vi "Alignment Value Change.vi"(8 "error in":errorcluster, 9 "NewVal":T1 items=["left", "center", "right"], 11 "Line Text":refnum<vi>[](array[refnum])) -> (0 "error out":errorcluster)   [LabVIEW 2020]
uses:
  vi.lib/LabVIEW Icon API/lv_icon/Controls/Alignment.ctl
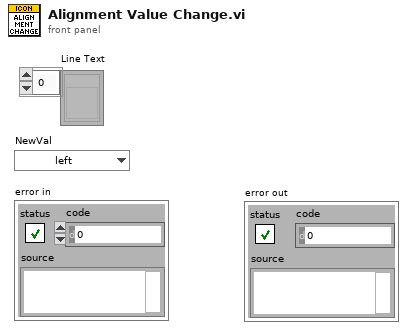
[diagram p1: front panel]
types:
  T1 = typedef "Alignment.ctl" = u16
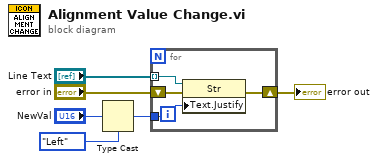
[diagram p0: block diagram]
diagram:
  n1 = Type Cast(type=enum16{"Left", "Center", "Right"}."Left" ("Text.Justification"), x="NewVal") -> (*(type *) &x=w3:enum16{"Left", "Center", "Right"})
  n2 = for {
    shift-right: [w9] -> w6
    shift-left: "error in" -> [w10]
    tunnel: "Line Text" -> [w8] mode=indexing
    tunnel: w3 -> [w7]
    n3 = property class="Str"(reference=w8, error in=w10, "Text.Justify"=w7) -> (error out=w9:errorcluster)  [unwired: 1 out]
  }
  "error out" <- w6
